vi "Read Stream State.vi"(8 "error in":errorcluster, 9 "request id":string, 10 "cancelled":refnum<queue>, 11 "stream key":string) -> (0 "error out":errorcluster, 1 "last probe":u32, 2 "last progress":dbl, 3 "cancelled?":bool)   [LabVIEW 2020, in "MCP Server.lvlib"]
doc: "Reads what is known about the streamed tools/call that is running, for Report Progress.vi and Cancel Requested.vi.\n\ncancelled? is TRUE when the request has been cancelled: the state stored by Stream State.vi says so for this stream, the client closed the stream (the cancelled flag queue of its MCP SSE Response holds TRUE), or (legacy) the client sent notifications/cancelled with the id of this request (Legacy Cancellations.vi).\n\nlast progress and last probe come from the state stored for this stream (stream key): the last progress value sent and the tick count (ms) of the last event or probe. A state stored for another stream is ignored: then last progress is NaN and last probe is 0.\n\nOutside a streamed request (stream key empty) only the legacy cancellation counts. Runs regardless of error in, which is passed through unchanged; errors of the reads are not passed on."
uses:
  MCP Server.lvlib
  20a4fcc1-f35a-4030-95e7-aedd8664271a.vi
  9b3dc396-53b4-4123-8340-9a1c69792bfa.vi
  e952fec2-39d2-4f94-8188-1a3d85b25364.vi
  <vilib>/JDP Science/JSONtext/Next JSON Value.vi
  <vilib>/JDP Science/JSONtext/String Subset.vi
  <vilib>/JDP Science/JSONtext/Parsing/Advance past next JSON Value (inlined COPY).vi
  <vilib>/JDP Science/JSONtext/Parsing/Advance past whitespace.vi
  <vilib>/JDP Science/JSONtext/Parsing/Advance past String.vi
  <vilib>/JDP Science/JSONtext/Parsing/Advance past Number.vi
  <vilib>/JDP Science/JSONtext/Parsing/Advance past Line Ending.vi
  <vilib>/JDP Science/JSONtext/Variant to JSON Text.vi
  <vilib>/JDP Science/JSONtext/Parsing/Parse Full Path or Item Name.vi
  <vilib>/JDP Science/JSONtext/Parsing/Advance past Array.vi
  <vilib>/JDP Science/JSONtext/Parsing/Advance past Object.vi
  <vilib>/JDP Science/JSONtext/support/Error Cluster From Code.vi
  <vilib>/JDP Science/JSONtext/Offset/Find Item Locations by Path.vi
  <vilib>/JDP Science/JSONtext/JSON text to Variant.vi
  <vilib>/JDP Science/JSONtext/LVClass Serializer/JSONtext LVClass Serializer.lvclass
  <vilib>/JDP Science/JSONtext/JSONtext.lvlib
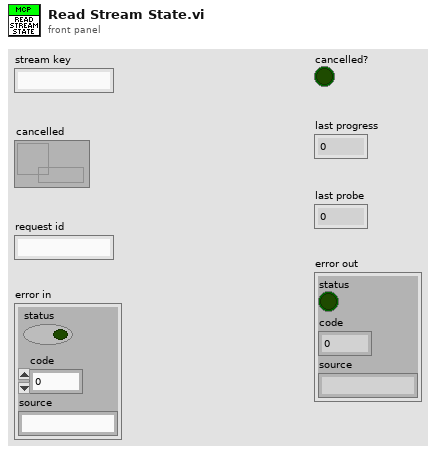
[diagram p1: front panel]
types:
  T1 = typedef "JSONtext.lvlib/JSON Value Type.ctl" = enum16{"Not a JSON Value", "JSON Object", "JSON Array", "String", "Number", "true", "false", "null"}
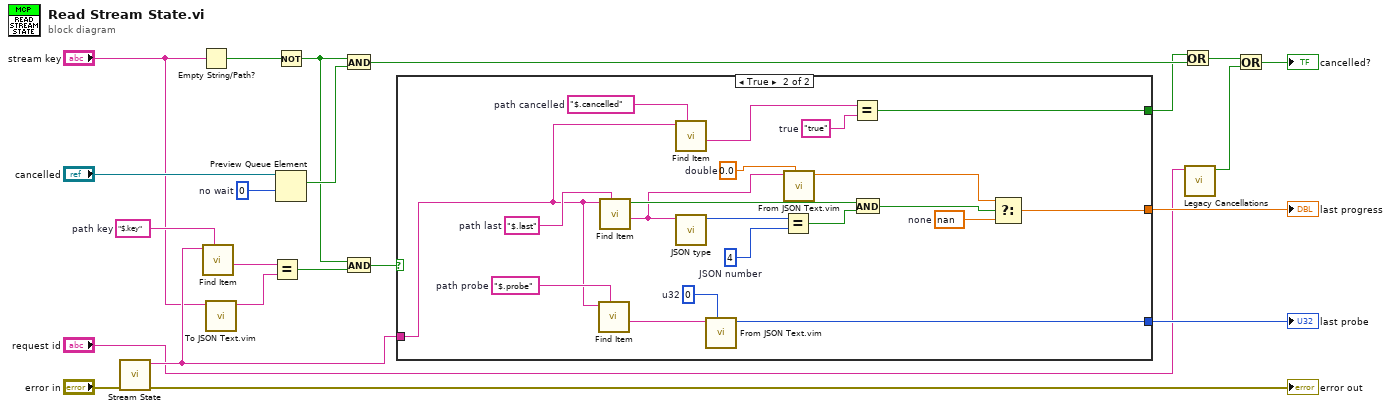
[diagram p0: block diagram]
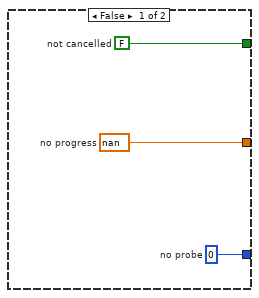
[diagram p2: hidden frame]
diagram:
  w6 = 0  # no wait
  w5 = "$.key"  # path key
  n1 = call "Stream State.vi"("error in"="error in") -> ("error out"=→"error out":errorcluster, "state out"=w11:string)  [unwired: 9 in]
  n2 = Empty String/Path?(string/path="stream key") -> (empty?=w12:bool)
  n3 = call <vilib>:"Find Item.vi"("$Path or Item Name"=w5, "JSON"=w11) -> ("<JSON>"=w15:string)  [unwired: 6 in, 3 out]
  n4 = call "To JSON Text.vim"("Anything"="stream key") -> ("<JSON>"=w14:string)  [unwired: 9 in, 1 out]
  n5 = Equal?(x=w15, y=w14) -> (x = y?=w16:bool)
  n6 = Not(x=w12) -> (.not. x?=w13:bool)
  n7 = Preview Queue Element(queue="cancelled", timeout in ms (-1)=w6) -> (element=w19:bool)  [unwired: 1 in, 3 out]
  n8 = And(x=w13, y=w19) -> (x .and. y?=w20:bool)
  n9 = And(x=w13, y=w16) -> (x .and. y?=w17:bool)
  n10 = case shown="True" w17 {
    tunnel: w11 -> [_ w26]
    tunnel: [w23 w27] -> w18
    tunnel: [w25 w29] -> w9
    tunnel: [w24 w28] -> w8
    frame False {
      w25 = u32 0  # no probe
      w24 = nan  # no progress
      w23 = FALSE  # not cancelled
    }
    frame True {
      w37 = u32 0  # u32
      w36 = nan  # none
      w35 = u16 4  # JSON number
      w34 = 0.0  # double
      w33 = "true"  # true
      w32 = "$.probe"  # path probe
      w31 = "$.last"  # path last
      w30 = "$.cancelled"  # path cancelled
      n11 = call <vilib>:"Find Item.vi"("$Path or Item Name"=w32, "JSON"=w26) -> ("<JSON>"=w45:string)  [unwired: 6 in, 3 out]
      n12 = call <vilib>:"Find Item.vi"("$Path or Item Name"=w31, "JSON"=w26) -> ("<JSON>"=w39:string, "Found"=w40:bool)  [unwired: 6 in, 2 out]
      n13 = call <vilib>:"Find Item.vi"("$Path or Item Name"=w30, "JSON"=w26) -> ("<JSON>"=w38:string)  [unwired: 6 in, 3 out]
      n14 = call <vilib>:"JSON type.vi"("JSON"=w39) -> ("JSON Value Type"=w41:T1)  [unwired: 9 in, 1 out]
      n15 = call "From JSON Text.vim"("Data Type and Default Value"=w37, "JSON"=w45) -> ("Data out"=w29:u32)  [unwired: 8 in, 1 out]
      n16 = Equal?(x=w41, y=w35) -> (x = y?=w42:bool)
      n17 = call "From JSON Text.vim"("Data Type and Default Value"=w34, "JSON"=w39) -> ("Data out"=w44:dbl)  [unwired: 8 in, 1 out]
      n18 = Equal?(x=w38, y=w33) -> (x = y?=w27:bool)
      n19 = And(x=w40, y=w42) -> (x .and. y?=w43:bool)
      n20 = Select(t=w44, s=w43, f=w36) -> (s? t:f=w28:dbl)
    }
  }
  "last progress" <- w8
  "last probe" <- w9
  n21 = Or(x=w18, y=w20) -> (x .or. y?=w22:bool)
  n22 = call "Legacy Cancellations.vi"("request id"="request id") -> ("recorded?"=w21:bool)  [unwired: 9 in, 1 out]
  n23 = Or(x=w22, y=w21) -> (x .or. y?=→"cancelled?":bool)
